vi "DISREADER.vi"() -> ()   [LabVIEW 2017]
panel:
  in  "stop":bool
  out "distance (m)":dbl
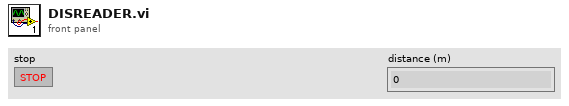
[diagram p1: front panel]
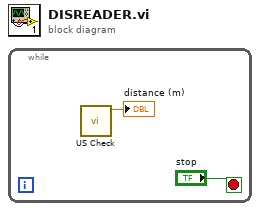
[diagram p0: block diagram]
diagram:
  n1 = while {
    stop <- "stop" stop-if-true
    n2 = call "US Check.vi"() -> ("distance (m)"=→"distance (m)":dbl)  [unwired: 11 in]
  }
